vi "Callback Change Direction.vi"(6 "Variant":variant, 8 "error in (no error)":errorcluster, 9 "old values":string[][](array[string]), 10 "object ref in":T2, 11 "Cluster":T3) -> (0 "error out":errorcluster)   [LabVIEW 2015, in "Scan Engine editor node.lvclass"]
uses:
  Scan Engine editor node.lvclass
  <vilib>/NI/DCAF/Tag Editor Core/Table API/Table Manager/Cell Change.ctl
  <vilib>/NI/DCAF/Tag Editor Core/Table API/Table Manager/object ref.ctl
  <vilib>/NI/DCAF/Tag Editor Core/Configuration Editor/Classes/Engine Parent/Engine Parent Editor Node.lvclass
  <vilib>/NI/DCAF/Tag Editor Core/Configuration Editor/Classes/Module editor node/module editor node.lvclass
  Permissions Enum.ctl
  configuration/Scan Engine configuration.lvclass
  <vilib>/NI/Module Execution Interface/Engine Configuration/engine configuration.lvclass
  configuration/Scan Engine configuration.lvclass/Scan Engine configuration.ctl
  <vilib>/NI/Tag Bus Module Framework/channel/TBM channel.lvclass/TBM channel.ctl
  <vilib>/NI/Configuration Framework/serializable configuration/NISE_CEF_serializable configuration.lvclass/NISE_CEF_serializable configuration.ctl
  <vilib>/Utility/LVClass/Get LV Class Name.vi
  <vilib>/NI/Configuration Framework/error generator/NISE_error generator.vi
  configuration/Get Line Name.vi
  configuration/Find Duplicate.vi
  <vilib>/Utility/error.llb/Error Cluster From Error Code.vi
  <vilib>/NI/Tag Bus Module Framework/channel/TBM channel.lvclass
  <vilib>/NI/DCAF/Tag Editor Core/Table API/Table Manager.lvlib
  <vilib>/NI/Configuration Framework/serializable configuration/NISE_CEF_serializable configuration.lvclass
  <vilib>/NI/DCAF/Tag Editor Core/Table API/Table Manager/Table Manager.lvclass
panel:
  in  "Permissions":T1
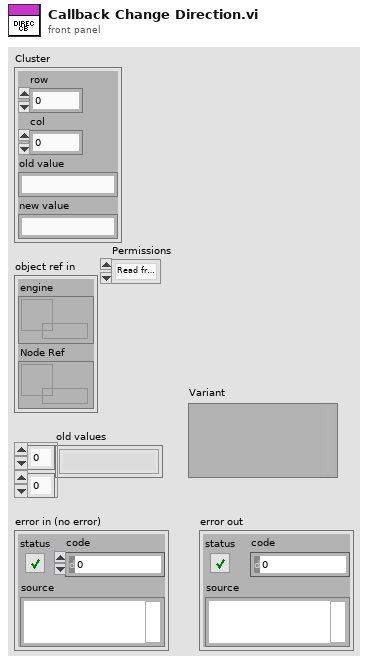
[diagram p1: front panel]
types:
  T1 = typedef "Scan Engine editor node.lvclass/Permissions Enum.ctl" = enum16{"Read from HW", "Write to HW"}
  T2 = typedef "Table Manager.lvlib/Table Manager.lvclass/object ref.ctl" = cluster{"engine":refnum<data-value>, "Node Ref":refnum<data-value>}
  T3 = typedef "Table Manager.lvlib/Cell Change.ctl" = cluster{"row":i32, "col":i32, "old value":string, "new value":string}
  T4 = typedef "TBM channel.lvclass/channel classification.ctl" = enum16{"input data", "output data", "processing parameter", "processing result"}
  T5 = typedef "Scan Engine configuration.lvclass/Line.ctl" = cluster{"channel":refnum<class "TBM channel.lvclass">, "Tag":string}
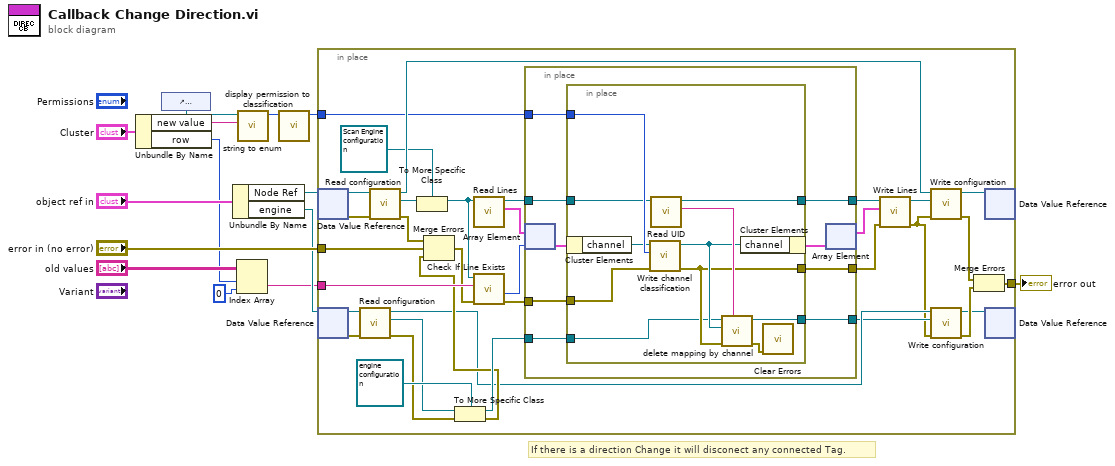
[diagram p0: block diagram]
diagram:
  # "If there is a direction Change it will disconect any connected Tag."
  n1 = Unbundle By Name("Cluster") -> ("new value"=w1:string, "row"=w2:i32)
  n2 = control-ref of="Permissions"() -> (w8:refnum<vi>)
  n3 = Unbundle By Name("object ref in") -> ("Node Ref"=w11:refnum<data-value>, "engine"=w10:refnum<data-value>)
  n4 = Index Array(array="old values", index (row)=w2, index (col)=0 ("disabled index (col)")) -> (element=w3:string)
  n5 = call <vilib>:"string to enum.vi"("String"=w1, "Enum"=w8) -> ("Value"=w7:i32)  [unwired: 8 in, 1 out]
  n6 = call "display permission to classification.vi"("display permissions"=w7) -> ("channel classification"=w6:T4)  [unwired: 10 in]
  n7 = in-place {
    in-place-border: [w46] -> w14
    in-place-border: "error in (no error)" -> [w27]
    in-place-border: w6 -> [w34]
    in-place-border: w3 -> [w33]
    n8 = in-place-dvr #1(w11) -> (w43:refnum<class "module editor node.lvclass">, w45:errorcluster)
    n9 = in-place-dvr #2(w10) -> (w26:refnum<class "Engine Parent Editor Node.lvclass">, w25:errorcluster)
    n10 = call-dynamic "Read configuration.vi"("error in"=w25, "NISE_CEF_serializable node in"=w26) -> ("error out"=w21:errorcluster, "configuration"=w23:refnum<class "NISE_CEF_serializable configuration.lvclass">, "NISE_CEF_serializable node out"=w19:refnum<class "Engine Parent Editor Node.lvclass">)  [unwired: 7 in]
    n11 = call-dynamic "Read configuration.vi"("error in"=w45, "NISE_CEF_serializable node in"=w43) -> ("error out"=w44:errorcluster, "configuration"=w41:refnum<class "NISE_CEF_serializable configuration.lvclass">, "NISE_CEF_serializable node out"=w42:refnum<class "module editor node.lvclass">)  [unwired: 7 in]
    n12 = To More Specific Class(target class=refnum<class "Scan Engine configuration.lvclass"> refnum ("tag bus configurable plugin module configuration"), reference=w41) -> (specific class reference=w38:refnum<class "Scan Engine configuration.lvclass">)  [unwired: 1 in, 1 out]
    n13 = To More Specific Class(target class=refnum<class "engine configuration.lvclass"> refnum ("engine configuration in"), reference=w23, error in=w21) -> (specific class reference=w22:refnum<class "engine configuration.lvclass">, error out=w20:errorcluster)
    n14 = Merge Errors(w44, w27, w20) -> (w30:errorcluster)
    n15 = call "Read Lines.vi"("Scan Engine configuration in"=w38) -> ("Lines"=w37:T5[], "Scan Engine configuration out"=w32:refnum<class "Scan Engine configuration.lvclass">)  [unwired: 8 in, 1 out]
    n16 = call-dynamic "Check If Line Exists.vi"("error in"=w30, "name to locate"=w33, "Scan Engine configuration in"=w38) -> ("error out"=w29:errorcluster, "index"=w35:i32)  [unwired: 4 in, 3 out]
    n17 = in-place {
      in-place-border: w34 -> [w55]
      in-place-border: w32 -> [w54]
      in-place-border: [w53] -> w31
      in-place-border: w22 -> [w52]
      in-place-border: [w51] -> w18
      in-place-border: w29 -> [w50]
      in-place-border: [w49] -> w28
      n18 = in-place-array #3(w37, w35) -> (w57:T5)
      n19 = in-place {
        in-place-border: w55 -> [w68]
        in-place-border: w54 -> [w67]
        in-place-border: [w66] -> w53
        in-place-border: w52 -> [w58]
        in-place-border: [w64] -> w51
        in-place-border: w50 -> [w61]
        in-place-border: [w59] -> w49
        n20 = in-place-cluster #4(w57) -> ("channel"=w65:refnum<class "TBM channel.lvclass">)
        n21 = call <vilib>:"Write channel classification.vi"("error in"=w61, "channel classification"=w68, "channel in"=w65) -> ("error out"=w59:errorcluster, "channel out"=w62:refnum<class "TBM channel.lvclass">)  [unwired: 7 in]
        n22 = call <vilib>:"Read UID.vi"("configuration in"=w67) -> ("instance id"=w63:string, "configuration out"=w66:refnum<class "Scan Engine configuration.lvclass">)  [unwired: 8 in, 1 out]
        n23 = call <vilib>:"delete mapping by channel.vi"("owner ID"=w63, "error in"=w59, "channel"=w62, "engine configuration in"=w58) -> ("error out"=w60:errorcluster, "engine configuration out"=w64:refnum<class "engine configuration.lvclass">)  [unwired: 6 in]
        n24 = in-place-cluster #4("channel"=w62) -> (w56:T5)
        n25 = call <vilib>:"Clear Errors.vi"("error in (no error)"=w60) -> ()  [unwired: 5 in, 2 out]
      }
      n26 = in-place-array #3(w56) -> (w36:T5[])  [unwired: 1 out]
    }
    n27 = call "Write Lines.vi"("error in (no error)"=w28, "Lines"=w36, "Scan Engine configuration in"=w31) -> ("error out"=w17:errorcluster, "Scan Engine configuration out"=w39:refnum<class "Scan Engine configuration.lvclass">)  [unwired: 7 in]
    n28 = call-dynamic "Write configuration.vi"("error in"=w17, "configuration"=w39, "NISE_CEF_serializable node in"=w42) -> ("error out"=w47:errorcluster, "NISE_CEF_serializable node out"=w48:refnum<class "module editor node.lvclass">)  [unwired: 7 in]
    n29 = call-dynamic "Write configuration.vi"("error in"=w17, "configuration"=w18, "NISE_CEF_serializable node in"=w19) -> ("error out"=w16:errorcluster, "NISE_CEF_serializable node out"=w15:refnum<class "Engine Parent Editor Node.lvclass">)  [unwired: 7 in]
    n30 = Merge Errors(w47, w16) -> (w46:errorcluster)
    n31 = in-place-dvr #1(w48) -> ()  [unwired: 2 out]
    n32 = in-place-dvr #2(w15) -> ()  [unwired: 2 out]
  }
  "error out" <- w14
